vi "ZM-CP-init.vi"(8 "error in (no error)":errorcluster, 11 "ZM-CP-MX-multi_protocol in":refnum<class "ZM-CP-MX-multi_protocol.lvclass">) -> (0 "error out":errorcluster, 3 "ZM-CP-MX-multi_protocol out":refnum<class "ZM-CP-MX-multi_protocol.lvclass">)   [LabVIEW 2020, in "ZM-CP-MX-multi_protocol.lvlib" / "ZM-CP-MX-multi_protocol.lvclass"]
doc: "Initialises the communication protocol (dynamic dispatch): writes opened = TRUE through the private accessor Write opened. This is the real default of the parent; a child overrides it, calls the parent and then runs its own hook."
uses:
  ZM-CP-MX-multi_protocol.lvclass
  ZM-CP-communication_protocol/ZM-CP-communication_protocol/ZM-CP-communication_protocol.lvclass
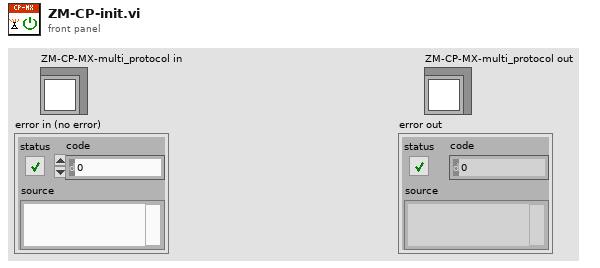
[diagram p1: front panel]
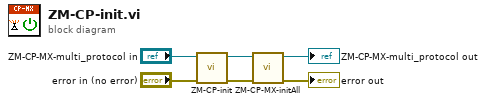
[diagram p0: block diagram]
diagram:
  n1 = call-parent "ZM-CP-init.vi"("error in (no error)"="error in (no error)", "ZM-CP-communication_protocol in"="ZM-CP-MX-multi_protocol in") -> ("error out"=w1:errorcluster, "ZM-CP-communication_protocol out"=w3:refnum<class "ZM-CP-MX-multi_protocol.lvclass">)  [unwired: 8 in]
  n2 = call "ZM-CP-MX-initAll.vi"("error in (no error)"=w1, "ZM-CP-communication_protocol in"=w3) -> ("error out"=→"error out":errorcluster, "ZM-CP-communication_protocol out"=→"ZM-CP-MX-multi_protocol out":refnum<class "ZM-CP-MX-multi_protocol.lvclass">)  [unwired: 8 in]
